vi "add.vi"(0 "reference":refnum<class "SequenceDiagramGraph.lvclass">, 1 "node":refnum<class "AbstractNode.lvclass">, 2 "point":T1 {"y" format="%.2f"; "x" format="%.2f"}, 5 "error in (no error)":errorcluster) -> (14 "reference out":refnum<class "SequenceDiagramGraph.lvclass">, 15 "added":bool, 19 "error out":errorcluster)   [LabVIEW 2020, in "SequenceDiagramGraph.lvclass"]
uses:
  <resource>/Framework/Providers/Open_GDS/UML/SequenceDiagramGraph_class/SequenceDiagramGraph.lvclass
  C:/Program Files (x86)/National Instruments/LabVIEW 2020/resource/Framework/Providers/Open_GDS/UML/Graph_class/Graph.lvclass
  <resource>/Framework/Providers/Open_GDS/UML/AbstractNode_class/AbstractNode.lvclass
  <resource>/Framework/Providers/Open_GDS/UML/General/Point/Point Point2D.ctl
  <resource>/Framework/Providers/Open_GDS/UML/CallNode_class/CallNode.lvclass
  <resource>/Framework/Providers/Open_GDS/UML/Graph_class/Graph.lvclass
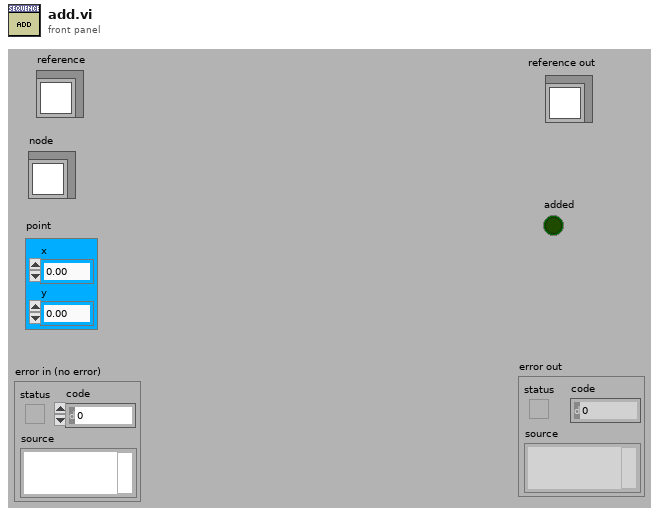
[diagram p1: front panel]
types:
  T1 = typedef "Point Point2D.ctl" = cluster{"x":dbl, "y":dbl}
  T2 = typedef "Graph.lvclass/ObjectAttributes.ctl" = cluster{"nodes":refnum<class "AbstractNode.lvclass">[], "edges":refnum<class "AbstractEdge.lvclass">[], "nodesToBeRemoved":refnum<class "AbstractNode.lvclass">[], "edgesToBeRemoved":refnum<class "AbstractEdge.lvclass">[], "needsLayout":bool, "LayoutNodes":refnum<class "AbstractNode.lvclass">[]}
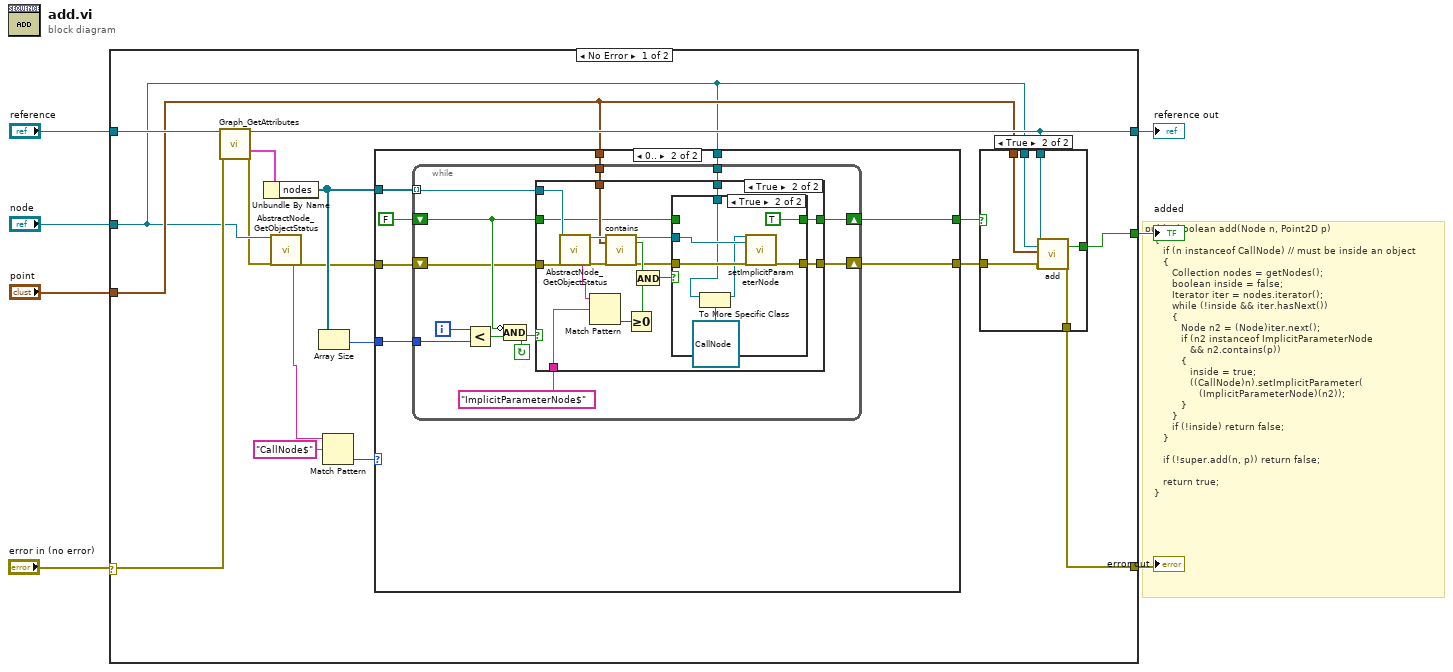
[diagram p0: block diagram]
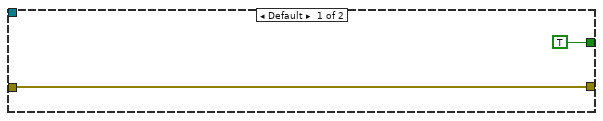
[diagram p3: hidden frame]
diagram:
  # "public boolean add(Node n, Point2D p)\n   {\n      if (n instanceof CallNode) // must be inside an object\n      {\n         Collection nodes = getNodes();\n         boolean inside = false;\n         Iterator iter = nodes.iterator();\n         while (!inside && iter.hasNext())\n         {\n            Node n2 = (Node)iter.next();\n            if (n2 instanceof ImplicitParameterNode\n               && n2.contains(p)) \n            {\n               inside = true;\n               ((CallNode)n).setImplicitParameter(\n                  (ImplicitParameterNode)(n2));\n            }\n         }\n         if (!inside) return false;\n      }\n\n      if (!super.add(n, p)) return false;\n\n      return true;\n   }"
  n1 = case shown="No Error" "error in (no error)" {
    selector: "error in (no error)" -> [w21 w83]
    tunnel: "reference" -> [w24 w84]
    tunnel: [w23 w83] -> w6
    tunnel: [w22 w84] -> w5
    tunnel: "node" -> [w18 _]
    tunnel: "point" -> [w19 _]
    tunnel: [w20 _] -> w1
    frame No Error {
      n2 = call <resource>:"Graph_GetAttributes.vi"("reference in"=w24, "error in (no error)"=w21) -> ("reference out"=w22:refnum<class "SequenceDiagramGraph.lvclass">, "Data"=w9:T2, "error out"=w15:errorcluster)  [unwired: 14 in, 1 out]
      n3 = Unbundle By Name(w9) -> ("nodes"=w14:refnum<class "AbstractNode.lvclass">[])
      n4 = call <resource>:"AbstractNode_GetObjectStatus.vi"("reference in"=w18, "error in (no error)"=w15) -> ("Class name"=w8:string, "error out"=w11:errorcluster)  [unwired: 16 out]
      n5 = Array Size(array=w14) -> (size(s)=w13:i32)
      n6 = Match Pattern(string=w8, regular expression="CallNode$") -> (offset past match=w16:i32)  [unwired: 4 out]
      n7 = case shown="0.." w16 {
        tunnel: w14 -> [_ w41]
        tunnel: w13 -> [_ w40]
        tunnel: w19 -> [_ w39]
        tunnel: [TRUE w38] -> w12
        tunnel: w18 -> [_ w37]
        tunnel: w11 -> [w34 w35]
        tunnel: [w34 w36] -> w10
        frame Default {
        }
        frame 0.. {
          n8 = while {
            shift-right: [w49] -> w38
            shift-left: FALSE -> [w50]
            tunnel: w41 -> [w48] mode=indexing
            tunnel: w40 -> [w53]
            tunnel: w39 -> [w46]
            tunnel: w37 -> [w45]
            shift-right: [w44] -> w36
            shift-left: w35 -> [w43]
            i -> [w54]
            stop <- w51 continue-if-true
            n9 = Less?(x=w54, y=w53) -> (x < y?=w52:bool)
            n10 = Compound Arithmetic op=AND(invert w50, w52) -> (w51:bool)
            n11 = case shown="True" w51 {
              tunnel: w50 -> [w56 w64]
              tunnel: [w56 w63] -> w49
              tunnel: w48 -> [_ w73]
              tunnel: "ImplicitParameterNode$" ("regular expression") -> [_ w72]
              tunnel: w46 -> [_ w68]
              tunnel: w45 -> [_ w60]
              tunnel: w43 -> [w55 w59]
              tunnel: [w55 w58] -> w44
              frame False {
              }
              frame True {
                n12 = call <resource>:"AbstractNode_GetObjectStatus.vi"("reference in"=w73, "error in (no error)"=w59) -> ("Class name"=w57:string, "reference out"=w70:refnum<class "AbstractNode.lvclass">, "error out"=w69:errorcluster)  [unwired: 15 out]
                n13 = Match Pattern(string=w57, regular expression=w72) -> (offset past match=w71:i32)  [unwired: 4 out]
                n14 = call-dynamic "contains.vi"("reference"=w70, "point2D"=w68, "error in (no error)"=w69) -> ("reference out"=w61:refnum<class "AbstractNode.lvclass">, "contains"=w66:bool, "error out"=w62:errorcluster)  [unwired: 14 in]
                n15 = Greater Or Equal To 0?(x=w71) -> (x >= 0?=w65:bool)
                n16 = And(x=w66, y=w65) -> (x .and. y?=w67:bool)
                n17 = case shown="True" w67 {
                  tunnel: w64 -> [w75 _]
                  tunnel: [w75 TRUE] -> w63
                  tunnel: w62 -> [w74 w81]
                  tunnel: w61 -> [_ w80]
                  tunnel: w60 -> [_ w78]
                  tunnel: [w74 w79] -> w58
                  frame False {
                  }
                  frame True {
                    n18 = To More Specific Class(target class=refnum<class "CallNode.lvclass"> refnum ("reference"), reference=w78) -> (specific class reference=w76:refnum<class "CallNode.lvclass">)  [unwired: 1 in, 1 out]
                    n19 = call-dynamic "setImplicitParameterNode.vi"("reference"=w76, "objectCallNodeRef"=w80, "error in (no error)"=w81) -> ("error out"=w79:errorcluster)  [unwired: 15 in, 1 out]
                  }
                }
              }
            }
          }
        }
      }
      n20 = case shown="True" w12 {
        selector: w12 -> [w26 _]
        tunnel: w18 -> [_ w31]
        tunnel: [w26 w27] -> w20
        tunnel: [w25 w28] -> w23
        tunnel: w19 -> [_ w30]
        tunnel: w10 -> [w25 w29]
        tunnel: w22 -> [_ w32]
        frame False {
        }
        frame True {
          n21 = call-parent "add.vi"("reference"=w32, "node"=w31, "point"=w30, "error in (no error)"=w29) -> ("added"=w27:bool, "error out"=w28:errorcluster)  [unwired: 13 in, 1 out]
        }
      }
    }
    frame Error {
    }
  }
  "reference out" <- w5
  "error out" <- w6
  "added" <- w1
